vi "Create LV File.vi"(6 "Output Folder":path, 8 "error in":errorcluster, 9 "Template":path, 10 "ILabVIEW File":refnum<class "ILabVIEW File.lvclass">, 11 "ILV File Creator in":refnum<class "ILV File Creator.lvclass">) -> (0 "error out":errorcluster, 2 "File Path":path, 3 "ILV File Creator out":refnum<class "ILV File Creator.lvclass">)   [LabVIEW 2026, in "ILV File Creator.lvclass"]
doc: "Create labview file."
uses:
  ILV File Creator.lvclass
  ILabVIEW File/ILabVIEW File.lvclass
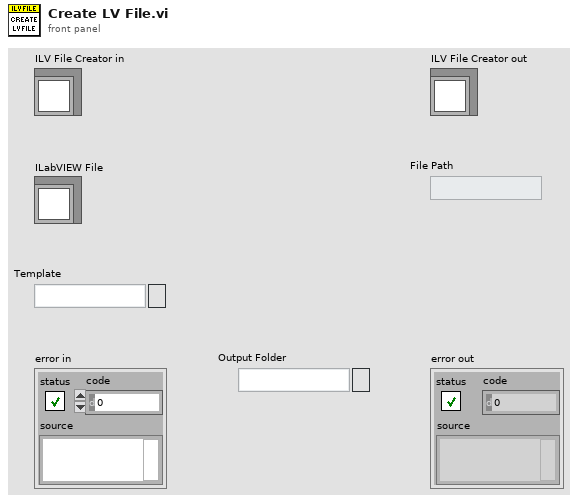
[diagram p1: front panel]
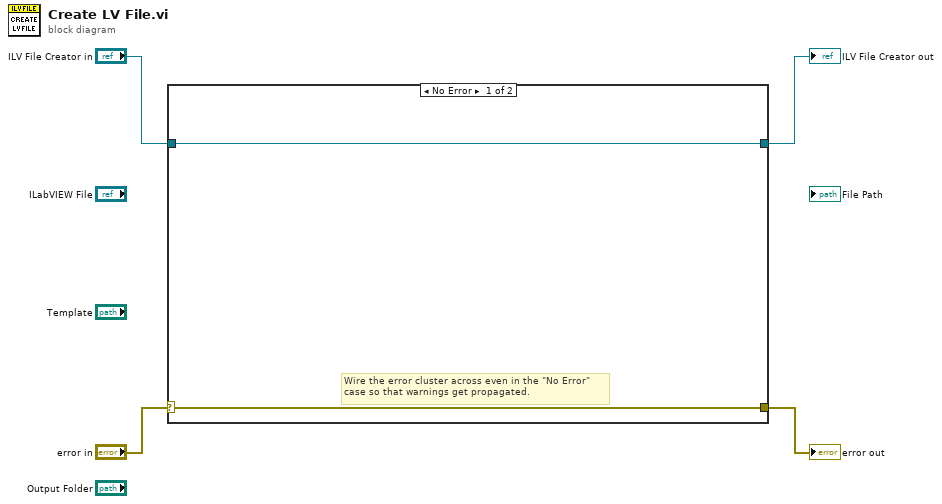
[diagram p0: block diagram]
diagram:
  n1 = case shown="No Error" "error in" {
    selector: "error in" -> [w6 w8]
    tunnel: [w6 w8] -> w3
    tunnel: [w5 w7] -> w1
    tunnel: "ILV File Creator in" -> [w5 w7]
    frame No Error {
      # "Wire the error cluster across even in the \"No Error\"\ncase so that warnings get propagated."
    }
    frame Error {
    }
  }
  "error out" <- w3
  "ILV File Creator out" <- w1
